vi "AI.Range to String.vi"(11 "AI.Range":T1) -> (3 "string":string)   [LabVIEW 2019, in "Instrument.Lockin.lvlib" / "Instrument.Lockin.lvclass"]
uses:
  Instrument.Lockin.lvclass
  Lockin.Typedefs/DAQ/DAQ.Config.AI.Range--enum.ctl
  Lockin.Typedefs/Lockin.Typedefs.lvlib
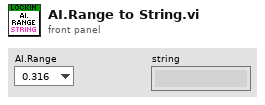
[diagram p1: front panel]
types:
  T1 = typedef "Lockin.Typedefs.lvlib/DAQ.Config.AI.Range--enum.ctl" = enum16{"0.316", "1.00", "3.16", "10.0", "31.6", "42.4", ""}
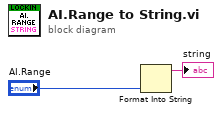
[diagram p0: block diagram]
diagram:
  n1 = Format Into String("AI.Range") -> (resulting string=→"string":string)  [unwired: 3 in, 1 out]
